vi "VIH Project - New Project - Master Rule (JS Based).vi"(8 "error in":errorcluster) -> (0 "error out":errorcluster, 3 "Master Rule":T1)   [LabVIEW 2014]
doc: "::: VI Helpeks :::\nCopyright (c) 2000-2026 Konstantin Shifershteyn. All rights reserved."
uses:
  _VIH HelpGen.llb/VIH HelpGen Typedef - Cluster - Group Rule.ctl
  _VIH HelpGen.llb/VIH HelpGen Typedef - Enum - Default,Enable,Disable.ctl
  _VIH HelpGen.llb/VIH HelpGen Typedef - Cluster - Group Rule - Source Paths.ctl
  _VIH HelpGen.llb/VIH HelpGen Typedef - Cluster - Group Rule - Target Paths.ctl
  _VIH HelpGen.llb/VIH HelpGen Typedef - Enum - Description Mode.ctl
  _VIH HelpGen.llb/VIH HelpGen Typedef - Cluster - Control Rule.ctl
  _VIH HelpGen.llb/VIH HelpGen Typedef - Cluster - Enum Value Info.ctl
  _VIH HelpGen.llb/VIH HelpGen Typedef - Cluster - Group Rule - Flags.ctl
panel:
  # "VI Helpeks\nCopyright (c) 2012-2026 Konstantin Shifershteyn"
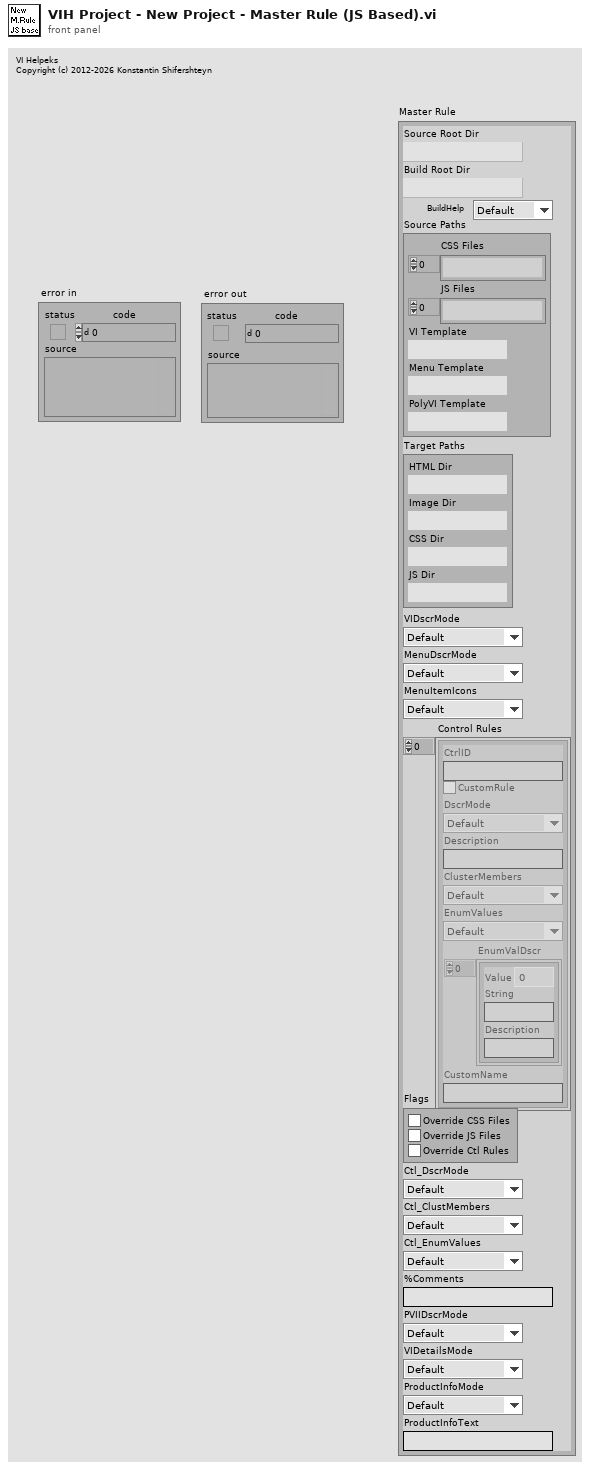
[diagram p1: front panel]
types:
  T1 = typedef "VIH HelpGen Typedef - Cluster - Group Rule.ctl" = cluster{"Source Root Dir":path, "Build Root Dir":path, "BuildHelp":T2, "Source Paths":T3, "Target Paths":T4, "VIDscrMode":T5, "MenuDscrMode":T5, "MenuItemIcons":T2, "Control Rules":T6[], "Flags":T8, "Ctl_DscrMode":T5, "Ctl_ClustMembers":T2, "Ctl_EnumValues":T2, "%Comments":string, "PVIIDscrMode":T5, "VIDetailsMode":T5, "ProductInfoMode":T2, "ProductInfoText":string}
  T2 = typedef "VIH HelpGen Typedef - Enum - Default,Enable,Disable.ctl" = enum16{"Default", "Enable", "Disable"}
  T3 = typedef "VIH HelpGen Typedef - Cluster - Group Rule - Source Paths.ctl" = cluster{"CSS Files":path[], "JS Files":path[], "VI Template":path, "Menu Template":path, "PolyVI Template":path}
  T4 = typedef "VIH HelpGen Typedef - Cluster - Group Rule - Target Paths.ctl" = cluster{"HTML Dir":path, "Image Dir":path, "CSS Dir":path, "JS Dir":path}
  T5 = typedef "VIH HelpGen Typedef - Enum - Description Mode.ctl" = enum16{"Default", "Description", "Description1", "Description2", "Custom", "None"}
  T6 = typedef "VIH HelpGen Typedef - Cluster - Control Rule.ctl" = cluster{"CtrlID":string, "CustomRule":bool, "DscrMode":T5, "Description":string, "ClusterMembers":T2, "EnumValues":T2, "EnumValDscr":T7[], "CustomName":string}
  T7 = typedef "VIH HelpGen Typedef - Cluster - Enum Value Info.ctl" = cluster{"Value":ext, "String":string, "Description":string}
  T8 = typedef "VIH HelpGen Typedef - Cluster - Group Rule - Flags.ctl" = cluster{"Override CSS Files":bool, "Override JS Files":bool, "Override Ctl Rules":bool}
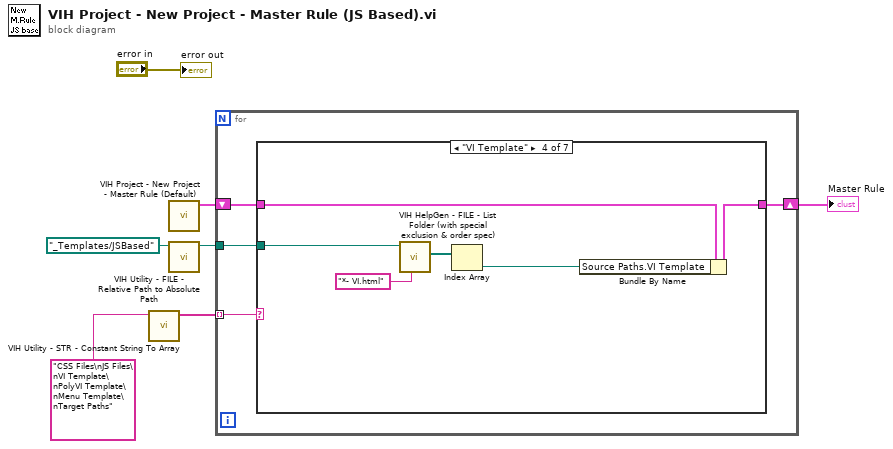
[diagram p0: block diagram]
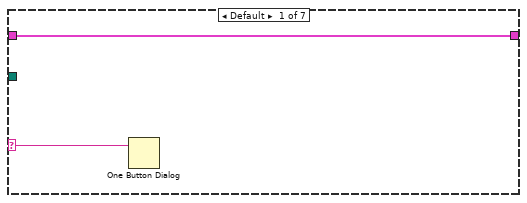
[diagram p2: hidden frame]
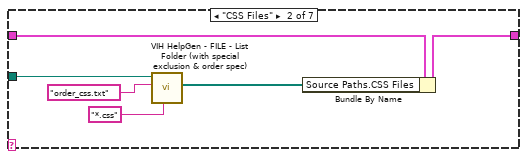
[diagram p3: hidden frame]
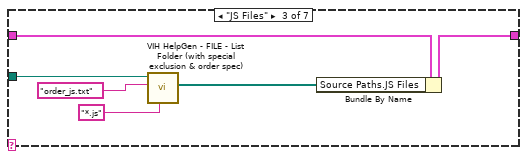
[diagram p4: hidden frame]
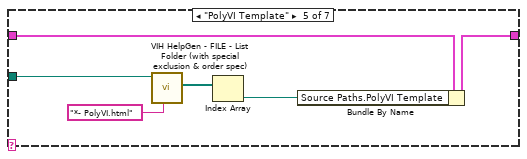
[diagram p5: hidden frame]
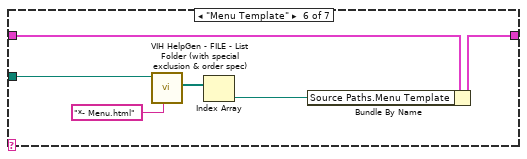
[diagram p6: hidden frame]
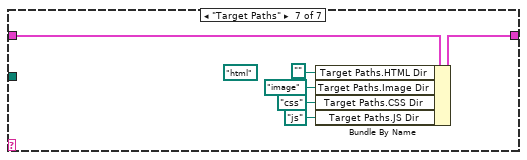
[diagram p7: hidden frame]
diagram:
  n1 = call "VIH Utility - STR - Constant String To Array.vi"("String in"="CSS Files\nJS Files\nVI Template\nPolyVI Template\nMenu Template\nTarget Paths") -> ("Array out"=w6:string[])  [unwired: 10 in]
  n2 = call "VIH Project - New Project - Master Rule (Default).vi"() -> ("Master Rule"=w1:T1)  [unwired: 10 in, 1 out]
  n3 = call "VIH Utility - FILE - Relative Path to Absolute Path.vi"("Path"=path "_Templates/JSBased") -> ("Path out"=w3:path)  [unwired: 9 in, 1 out]
  n4 = for {
    shift-right: [w11] -> w2
    shift-left: w1 -> [w10]
    tunnel: w6 -> [w9] mode=indexing
    tunnel: w3 -> [w8]
    n5 = case shown="\"VI Template\"" w9 {
      selector: w9 -> [w12 _ _ _ _ _ _]
      tunnel: [w13 w19 w25 w31 w37 w43 w49] -> w11
      tunnel: w10 -> [w13 w18 w24 w30 w36 w42 w48]
      tunnel: w8 -> [_ w16 w22 w27 w33 w39 _]
      frame Default {
        n6 = One Button Dialog(message=w12) -> ()  [unwired: 1 in, 1 out]
      }
      frame "CSS Files" {
        n7 = call "VIH HelpGen - FILE - List Folder (with special exclusion & order spec).vi"("pattern"="*.css", "order file name"="order_css.txt", "path"=w16) -> ("File paths"=w15:path[])  [unwired: 6 in, 2 out]
        n8 = Bundle By Name(cluster=w18, "Source Paths.CSS Files"=w15) -> (w19:T1)
      }
      frame "JS Files" {
        n9 = call "VIH HelpGen - FILE - List Folder (with special exclusion & order spec).vi"("pattern"="*.js", "order file name"="order_js.txt", "path"=w22) -> ("File paths"=w21:path[])  [unwired: 6 in, 2 out]
        n10 = Bundle By Name(cluster=w24, "Source Paths.JS Files"=w21) -> (w25:T1)
      }
      frame "VI Template" {
        n11 = call "VIH HelpGen - FILE - List Folder (with special exclusion & order spec).vi"("pattern"="*- VI.html", "path"=w27) -> ("File paths"=w28:path[])  [unwired: 7 in, 2 out]
        n12 = Index Array(array=w28) -> (element=w26:path)  [unwired: 1 in]
        n13 = Bundle By Name(cluster=w30, "Source Paths.VI Template"=w26) -> (w31:T1)
      }
      frame "PolyVI Template" {
        n14 = call "VIH HelpGen - FILE - List Folder (with special exclusion & order spec).vi"("pattern"="*- PolyVI.html", "path"=w33) -> ("File paths"=w34:path[])  [unwired: 7 in, 2 out]
        n15 = Index Array(array=w34) -> (element=w32:path)  [unwired: 1 in]
        n16 = Bundle By Name(cluster=w36, "Source Paths.PolyVI Template"=w32) -> (w37:T1)
      }
      frame "Menu Template" {
        n17 = call "VIH HelpGen - FILE - List Folder (with special exclusion & order spec).vi"("pattern"="*- Menu.html", "path"=w39) -> ("File paths"=w40:path[])  [unwired: 7 in, 2 out]
        n18 = Index Array(array=w40) -> (element=w38:path)  [unwired: 1 in]
        n19 = Bundle By Name(cluster=w42, "Source Paths.Menu Template"=w38) -> (w43:T1)
      }
      frame "Target Paths" {
        (unwired) path "html" ("Target Paths.HTML Dir")
        n20 = Bundle By Name(cluster=w48, "Target Paths.HTML Dir"=path "", "Target Paths.Image Dir"=path "image", "Target Paths.CSS Dir"=path "css", "Target Paths.JS Dir"=path "js") -> (w49:T1)
      }
    }
  }
  "Master Rule" <- w2
  "error out" <- "error in"
